vi "Build Win32 Wrappers.vi"(0 "only these wrappers":string[](array[string]), 11 "error in":errorcluster) -> (4 "wrappers":path[](array[path]), 15 "error out":errorcluster)   [LabVIEW 2020]
doc: "Creates or overwrites the Win32 wrapper VIs of the RemoteVI toolkit in source\\Win32 by VI scripting - one VI per DLL function, each listed in the wrapper specs constant on this diagram (wrapper name, template, DLL, function, parameter lines, link lines - see W32B Parse Spec.vi for the line format, and UI thread?). Each wrapper starts as a copy of its template in scripts\\Win32 Wrapper Templates (front panel, connector pane, icon, descriptions, helper nodes), then gets a Call Library Function Node placed, configured (stdcall, run in any thread - or in LabVIEW's UI thread when the spec's UI thread? is TRUE, typed parameters) and wired by VI Server - the one node AIXML cannot author. only these wrappers limits the run to the named wrapper VIs (empty = all); a wrapper that is loaded in LabVIEW (called by a running VI) cannot be overwritten. Run it from the IDE whenever a template or a spec changes. Paths are found relative to this VI, so the repository may live anywhere. The AIXML sources of the templates are in tools\\aixml\\Win32."
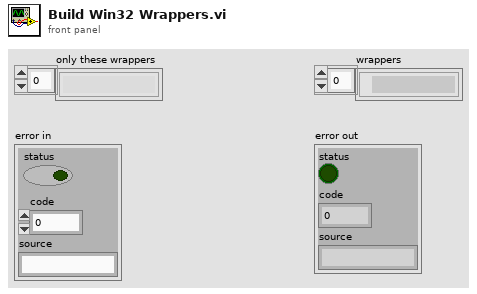
[diagram p1: front panel]
types:
  T1 = cluster{"wrapper name":string, "template":string, "library":path, "function":string, "parameters":string, "links":string, "UI thread?":bool}[]
  T2 = cluster{"function name":string, "library path":path, "parameter info":cluster{"Parameter Name":string, "Num Dimensions":i32, "Parameter Type":enum16{"Numeric", "Array", "String", "Waveform", "Digital Waveform", "Digital Table", "ActiveX", "Any", "Instance Data Pointer", "Void"}, "Numeric Type":enum16{"I8", "I16", "I32", "I64", "U8", "U16", "U32", "U64", "SGL", "DBL", "PTR INT", "PTR UINT"}, "Param Passing":enum16{"By Value", "Pointer To Value"}, "Array Passing":enum16{"Array Data Pointer", "Array Handle", "Array Handle Pointer"}, "String Passing":enum16{"C String Pointer", "Pascal String Pointer", "String Handle", "String Handle Pointer"}, "Adapt Format":enum16{"By Value", "Pointer To Value"}, "ActiveX Types":enum16{"ActiveX Variant Pointer", "IDispatch* Pointer", "IUnknown* Pointer"}, "Const (unused)":bool, "Minimum Size":string}[]}
  T3 = cluster{"CLFN terminal":i32, "control label":string, "node class":string, "node source?":bool}[]
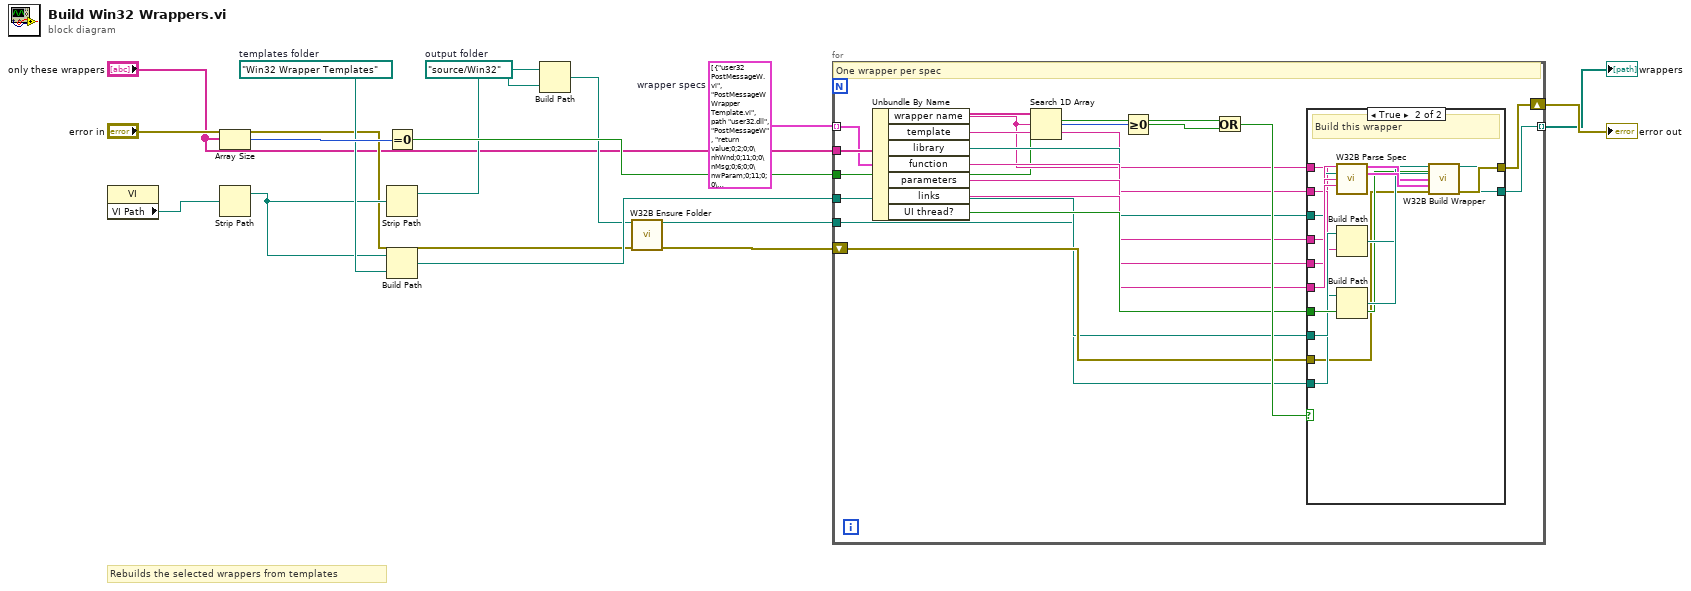
[diagram p0: block diagram]
diagram:
  w14 = T1 [{"wrapper name"="user32 PostMessageW.vi", "template"="PostMessageW Wrapper Template.vi", "library"=path "user32.dll", "function"="PostMessageW", "parameters"="return value;0;2;0;0\nhWnd;0;11;0;0\nMsg;0;6;0;0\nwParam;0;11;0;0\nlParam;0;10;0;0", "links"="2;error in (no error);;0\n3;error out;;0\n5;return value;;0\n6;hWnd;;0\n8;Msg;;0\n10;wParam;;0\n12;lParam;;0", "UI thread?"=FALSE}, {"wrapper name"="user32 ScreenToClient.vi", "template"="ScreenToClient Wrapper Template.vi", "library"=path "user32.dll", "function"="ScreenToClient", "parameters"="return value;0;2;0;0\nhWnd;0;11;0;0\nlpPoint;7;2;0;0", "links"="2;error in (no error);;0\n3;error out;;0\n5;return value;;0\n6;hWnd;;0\n8;;Bundler;1\n9;;Unbundler;0", "UI thread?"=FALSE}, {"wrapper name"="user32 FindWindowExW.vi", "template"="FindWindowExW Wrapper Template.vi", "library"=path "user32.dll", "function"="FindWindowExW", "parameters"="return value;0;11;0;0\nhWndParent;0;11;0;0\nhWndChildAfter;0;11;0;0\nlpszClass;1;5;0;0;1\nlpszWindow;1;5;0;0;1", "links"="2;error in;;0\n3;error out;;0\n5;hWnd;;0\n6;hWndParent;;0\n8;hWndChildAfter;;0\n10;lpszClass;;0\n12;lpszWindow;;0", "UI thread?"=FALSE}, {"wrapper name"="user32 GetWindowThreadProcessId.vi", "template"="GetWindowThreadProcessId Wrapper Template.vi", "library"=path "user32.dll", "function"="GetWindowThreadProcessId", "parameters"="return value;0;6;0;0\nhWnd;0;11;0;0\nlpdwProcessId;0;6;1;0", "links"="2;error in;;0\n3;error out;;0\n5;thread ID;;0\n6;hWnd;;0\n9;process ID;;0", "UI thread?"=FALSE}, {"wrapper name"="user32 IsWindowVisible.vi", "template"="IsWindowVisible Wrapper Template.vi", "library"=path "user32.dll", "function"="IsWindowVisible", "parameters"="return value;0;2;0;0\nhWnd;0;11;0;0", "links"="2;error in;;0\n3;error out;;0\n5;;Function;0\n6;hWnd;;0", "UI thread?"=FALSE}, {"wrapper name"="user32 IsIconic.vi", "template"="IsIconic Wrapper Template.vi", "library"=path "user32.dll", "function"="IsIconic", "parameters"="return value;0;2;0;0\nhWnd;0;11;0;0", "links"="2;error in;;0\n3;error out;;0\n5;;Function;0\n6;hWnd;;0", "UI thread?"=FALSE}, {"wrapper name"="user32 ShowWindow.vi", "template"="ShowWindow Wrapper Template.vi", "library"=path "user32.dll", "function"="ShowWindow", "parameters"="return value;0;2;0;0\nhWnd;0;11;0;0\nnCmdShow;0;2;0;0", "links"="2;error in;;0\n3;error out;;0\n5;return value;;0\n6;hWnd;;0\n8;nCmdShow;;0", "UI thread?"=FALSE}, {"wrapper name"="user32 GetWindowRect.vi", "template"="GetWindowRect Wrapper Template.vi", "library"=path "user32.dll", "function"="GetWindowRect", "parameters"="return value;0;2;0;0\nhWnd;0;11;0;0\nlpRect;7;2;0;0", "links"="2;error in;;0\n3;error out;;0\n5;return value;;0\n6;hWnd;;0\n8;;Bundler;1\n9;RECT;;0", "UI thread?"=FALSE}, {"wrapper name"="user32 GetClientRect.vi", "template"="GetClientRect Wrapper Template.vi", "library"=path "user32.dll", "function"="GetClientRect", "parameters"="return value;0;2;0;0\nhWnd;0;11;0;0\nlpRect;7;2;0;0", "links"="2;error in;;0\n3;error out;;0\n5;return value;;0\n6;hWnd;;0\n8;;Bundler;1\n9;RECT;;0", "UI thread?"=FALSE}, {"wrapper name"="user32 GetClassNameW.vi", "template"="GetClassNameW Wrapper Template.vi", "library"=path "user32.dll", "function"="GetClassNameW", "parameters"="return value;0;2;0;0\nhWnd;0;11;0;0\nlpClassName;1;5;0;0;1\nnMaxCount;0;2;0;0", "links"="2;error in;;0\n3;error out;;0\n5;return value;;0\n6;hWnd;;0\n8;;Unbundler;1\n9;;BuildArray;0\n10;nMaxCount;;0", "UI thread?"=FALSE}, {"wrapper name"="user32 GetWindowLongPtrW.vi", "template"="GetWindowLongPtrW Wrapper Template.vi", "library"=path "user32.dll", "function"="GetWindowLongPtrW", "parameters"="return value;0;10;0;0\nhWnd;0;11;0;0\nnIndex;0;2;0;0", "links"="2;error in;;0\n3;error out;;0\n5;return value;;0\n6;hWnd;;0\n8;nIndex;;0", "UI thread?"=FALSE}, {"wrapper name"="user32 SetWindowPos.vi", "template"="SetWindowPos Wrapper Template.vi", "library"=path "user32.dll", "function"="SetWindowPos", "parameters"="return value;0;2;0;0\nhWnd;0;11;0;0\nhWndInsertAfter;0;11;0;0\nX;0;2;0;0\nY;0;2;0;0\ncx;0;2;0;0\ncy;0;2;0;0\nuFlags;0;6;0;0", "links"="2;error in;;0\n3;error out;;0\n5;return value;;0\n6;hWnd;;0\n8;hWndInsertAfter;;0\n10;X;;0\n12;Y;;0\n14;cx;;0\n16;cy;;0\n18;uFlags;;0", "UI thread?"=FALSE}, {"wrapper name"="user32 SendMessageTimeoutW.vi", "template"="SendMessageTimeoutW Wrapper Template.vi", "library"=path "user32.dll", "function"="SendMessageTimeoutW", "parameters"="return value;0;10;0;0\nhWnd;0;11;0;0\nMsg;0;6;0;0\nwParam;0;11;0;0\nlParam;0;10;0;0\nfuFlags;0;6;0;0\nuTimeout;0;6;0;0\nlpdwResult;0;11;1;0", "links"="2;error in;;0\n3;error out;;0\n5;return value;;0\n6;hWnd;;0\n8;Msg;;0\n10;wParam;;0\n12;lParam;;0\n14;fuFlags;;0\n16;uTimeout;;0\n19;result;;0", "UI thread?"=FALSE}, {"wrapper name"="user32 GetDC.vi", "template"="GetDC Wrapper Template.vi", "library"=path "user32.dll", "function"="GetDC", "parameters"="return value;0;11;0;0\nhWnd;0;11;0;0", "links"="2;error in;;0\n3;error out;;0\n5;HDC;;0\n6;hWnd;;0", "UI thread?"=FALSE}, {"wrapper name"="user32 ReleaseDC.vi", "template"="ReleaseDC Wrapper Template.vi", "library"=path "user32.dll", "function"="ReleaseDC", "parameters"="return value;0;2;0;0\nhWnd;0;11;0;0\nhDC;0;11;0;0", "links"="2;error in;;0\n3;error out;;0\n5;return value;;0\n6;hWnd;;0\n8;hDC;;0", "UI thread?"=FALSE}, {"wrapper name"="kernel32 GetCurrentProcessId.vi", "template"="GetCurrentProcessId Wrapper Template.vi", "library"=path "kernel32.dll", "function"="GetCurrentProcessId", "parameters"="return value;0;6;0;0", "links"="2;error in;;0\n3;error out;;0\n5;process ID;;0", "UI thread?"=FALSE}, {"wrapper name"="gdi32 CreateCompatibleDC.vi", "template"="CreateCompatibleDC Wrapper Template.vi", "library"=path "gdi32.dll", "function"="CreateCompatibleDC", "parameters"="return value;0;11;0;0\nhdc;0;11;0;0", "links"="2;error in;;0\n3;error out;;0\n5;HDC;;0\n6;hdc;;0", "UI thread?"=FALSE}, {"wrapper name"="gdi32 CreateCompatibleBitmap.vi", "template"="CreateCompatibleBitmap Wrapper Template.vi", "library"=path "gdi32.dll", "function"="CreateCompatibleBitmap", "parameters"="return value;0;11;0;0\nhdc;0;11;0;0\ncx;0;2;0;0\ncy;0;2;0;0", "links"="2;error in;;0\n3;error out;;0\n5;HBITMAP;;0\n6;hdc;;0\n8;cx;;0\n10;cy;;0", "UI thread?"=FALSE}, {"wrapper name"="gdi32 SelectObject.vi", "template"="SelectObject Wrapper Template.vi", "library"=path "gdi32.dll", "function"="SelectObject", "parameters"="return value;0;11;0;0\nhdc;0;11;0;0\nh;0;11;0;0", "links"="2;error in;;0\n3;error out;;0\n5;previous object;;0\n6;hdc;;0\n8;h;;0", "UI thread?"=FALSE}, {"wrapper name"="gdi32 GetDIBits.vi", "template"="GetDIBits Wrapper Template.vi", "library"=path "gdi32.dll", "function"="GetDIBits", "parameters"="return value;0;2;0;0\nhdc;0;11;0;0\nhbm;0;11;0;0\nstart;0;6;0;0\ncLines;0;6;0;0\nlpvBits;1;6;0;0;1\nlpbmi;7;2;0;0\nusage;0;6;0;0", "links"="2;error in;;0\n3;error out;;0\n5;return value;;0\n6;hdc;;0\n8;hbm;;0\n10;start;;0\n12;cLines;;0\n14;lpvBits;;0\n15;lpvBits out;;0\n16;lpbmi;;0\n18;usage;;0", "UI thread?"=FALSE}, {"wrapper name"="gdi32 DeleteObject.vi", "template"="DeleteObject Wrapper Template.vi", "library"=path "gdi32.dll", "function"="DeleteObject", "parameters"="return value;0;2;0;0\nho;0;11;0;0", "links"="2;error in;;0\n3;error out;;0\n5;return value;;0\n6;ho;;0", "UI thread?"=FALSE}, {"wrapper name"="gdi32 DeleteDC.vi", "template"="DeleteDC Wrapper Template.vi", "library"=path "gdi32.dll", "function"="DeleteDC", "parameters"="return value;0;2;0;0\nhdc;0;11;0;0", "links"="2;error in;;0\n3;error out;;0\n5;return value;;0\n6;hdc;;0", "UI thread?"=FALSE}, {"wrapper name"="user32 PrintWindow.vi", "template"="PrintWindow Wrapper Template.vi", "library"=path "user32.dll", "function"="PrintWindow", "parameters"="return value;0;2;0;0\nhwnd;0;11;0;0\nhdcBlt;0;11;0;0\nnFlags;0;6;0;0", "links"="2;error in;;0\n3;error out;;0\n5;return value;;0\n6;hwnd;;0\n8;hdcBlt;;0\n10;nFlags;;0", "UI thread?"=FALSE}, {"wrapper name"="user32 SetWindowLongPtrW.vi", "template"="SetWindowLongPtrW Wrapper Template.vi", "library"=path "user32.dll", "function"="SetWindowLongPtrW", "parameters"="return value;0;10;0;0\nhWnd;0;11;0;0\nnIndex;0;2;0;0\ndwNewLong;0;10;0;0", "links"="2;error in;;0\n3;error out;;0\n5;return value;;0\n6;hWnd;;0\n8;nIndex;;0\n10;dwNewLong;;0", "UI thread?"=FALSE}, {"wrapper name"="user32 SetLayeredWindowAttributes.vi", "template"="SetLayeredWindowAttributes Wrapper Template.vi", "library"=path "user32.dll", "function"="SetLayeredWindowAttributes", "parameters"="return value;0;2;0;0\nhwnd;0;11;0;0\ncrKey;0;6;0;0\nbAlpha;0;4;0;0\ndwFlags;0;6;0;0", "links"="2;error in;;0\n3;error out;;0\n5;return value;;0\n6;hwnd;;0\n8;crKey;;0\n10;bAlpha;;0\n12;dwFlags;;0", "UI thread?"=FALSE}, {"wrapper name"="user32 GetCursorPos.vi", "template"="GetCursorPos Wrapper Template.vi", "library"=path "user32.dll", "function"="GetCursorPos", "parameters"="return value;0;2;0;0\nlpPoint;7;2;0;0", "links"="2;error in;;0\n3;error out;;0\n5;return value;;0\n6;;Bundler;1\n7;;Unbundler;0", "UI thread?"=FALSE}, {"wrapper name"="user32 GetKeyboardState.vi", "template"="GetKeyboardState Wrapper Template.vi", "library"=path "user32.dll", "function"="GetKeyboardState", "parameters"="return value;0;2;0;0\nlpKeyState;1;4;0;0;1", "links"="2;error in;;0\n3;error out;;0\n5;return value;;0\n6;;Unbundler;1\n7;;BuildArray;0", "UI thread?"=TRUE}, {"wrapper name"="user32 SetKeyboardState.vi", "template"="SetKeyboardState Wrapper Template.vi", "library"=path "user32.dll", "function"="SetKeyboardState", "parameters"="return value;0;2;0;0\nlpKeyState;1;4;0;0;1", "links"="2;error in;;0\n3;error out;;0\n5;return value;;0\n6;;Unbundler;1\n7;;BuildArray;0", "UI thread?"=TRUE}, {"wrapper name"="user32 GetGUIThreadInfo.vi", "template"="GetGUIThreadInfo Wrapper Template.vi", "library"=path "user32.dll", "function"="GetGUIThreadInfo", "parameters"="return value;0;2;0;0\nidThread;0;6;0;0\npgui;1;6;0;0;1", "links"="2;error in;;0\n3;error out;;0\n5;return value;;0\n6;thread ID;;0\n8;;Unbundler;1\n9;;BuildArray;0", "UI thread?"=FALSE}, {"wrapper name"="user32 GetSysColor.vi", "template"="GetSysColor Wrapper Template.vi", "library"=path "user32.dll", "function"="GetSysColor", "parameters"="return value;0;6;0;0\nnIndex;0;2;0;0", "links"="2;error in;;0\n3;error out;;0\n5;color;;0\n6;nIndex;;0", "UI thread?"=FALSE}, {"wrapper name"="user32 GetWindow.vi", "template"="GetWindow Wrapper Template.vi", "library"=path "user32.dll", "function"="GetWindow", "parameters"="return value;0;11;0;0\nhWnd;0;11;0;0\nuCmd;0;6;0;0", "links"="2;error in;;0\n3;error out;;0\n5;window;;0\n6;hWnd;;0\n8;uCmd;;0", "UI thread?"=FALSE}, {"wrapper name"="user32 GetAncestor.vi", "template"="GetAncestor Wrapper Template.vi", "library"=path "user32.dll", "function"="GetAncestor", "parameters"="return value;0;11;0;0\nhwnd;0;11;0;0\ngaFlags;0;6;0;0", "links"="2;error in;;0\n3;error out;;0\n5;ancestor;;0\n6;hwnd;;0\n8;gaFlags;;0", "UI thread?"=FALSE}, {"wrapper name"="user32 IsWindowEnabled.vi", "template"="IsWindowEnabled Wrapper Template.vi", "library"=path "user32.dll", "function"="IsWindowEnabled", "parameters"="return value;0;2;0;0\nhWnd;0;11;0;0", "links"="2;error in;;0\n3;error out;;0\n5;;Function;0\n6;hWnd;;0", "UI thread?"=FALSE}, {"wrapper name"="user32 GetWindowTextW.vi", "template"="GetWindowTextW Wrapper Template.vi", "library"=path "user32.dll", "function"="GetWindowTextW", "parameters"="return value;0;2;0;0\nhWnd;0;11;0;0\nlpString;1;5;0;0;1\nnMaxCount;0;2;0;0", "links"="2;error in;;0\n3;error out;;0\n5;return value;;0\n6;hWnd;;0\n8;;Unbundler;1\n9;;BuildArray;0\n10;nMaxCount;;0", "UI thread?"=FALSE}, {"wrapper name"="user32 ChildWindowFromPointEx.vi", "template"="ChildWindowFromPointEx Wrapper Template.vi", "library"=path "user32.dll", "function"="ChildWindowFromPointEx", "parameters"="return value;0;11;0;0\nhwnd;0;11;0;0\npt;0;7;0;0\nflags;0;6;0;0", "links"="2;error in;;0\n3;error out;;0\n5;child;;0\n6;hwnd;;0\n8;pt;;0\n10;flags;;0", "UI thread?"=FALSE}, {"wrapper name"="gdi32 CreateRectRgn.vi", "template"="CreateRectRgn Wrapper Template.vi", "library"=path "gdi32.dll", "function"="CreateRectRgn", "parameters"="return value;0;11;0;0\nx1;0;2;0;0\ny1;0;2;0;0\nx2;0;2;0;0\ny2;0;2;0;0", "links"="2;error in;;0\n3;error out;;0\n5;HRGN;;0\n6;x1;;0\n8;y1;;0\n10;x2;;0\n12;y2;;0", "UI thread?"=FALSE}, {"wrapper name"="user32 SetWindowRgn.vi", "template"="SetWindowRgn Wrapper Template.vi", "library"=path "user32.dll", "function"="SetWindowRgn", "parameters"="return value;0;2;0;0\nhWnd;0;11;0;0\nhRgn;0;11;0;0\nbRedraw;0;2;0;0", "links"="2;error in;;0\n3;error out;;0\n5;return value;;0\n6;hWnd;;0\n8;hRgn;;0\n10;bRedraw;;0", "UI thread?"=FALSE}, {"wrapper name"="gdi32 BitBlt.vi", "template"="BitBlt Wrapper Template.vi", "library"=path "gdi32.dll", "function"="BitBlt", "parameters"="return value;0;2;0;0\nhdc;0;11;0;0\nx;0;2;0;0\ny;0;2;0;0\ncx;0;2;0;0\ncy;0;2;0;0\nhdcSrc;0;11;0;0\nx1;0;2;0;0\ny1;0;2;0;0\nrop;0;6;0;0", "links"="2;error in;;0\n3;error out;;0\n5;return value;;0\n6;hdc;;0\n8;x;;0\n10;y;;0\n12;cx;;0\n14;cy;;0\n16;hdcSrc;;0\n18;x1;;0\n20;y1;;0\n22;rop;;0", "UI thread?"=FALSE}, {"wrapper name"="bcrypt BCryptGenRandom.vi", "template"="BCryptGenRandom Wrapper Template.vi", "library"=path "bcrypt.dll", "function"="BCryptGenRandom", "parameters"="return value;0;2;0;0\nhAlgorithm;0;11;0;0\npbBuffer;1;4;0;0;1\ncbBuffer;0;6;0;0\ndwFlags;0;6;0;0", "links"="2;error in;;0\n3;error out;;0\n5;return value;;0\n6;hAlgorithm;;0\n8;;Unbundler;1\n9;;BuildArray;0\n10;byte count;;0\n12;dwFlags;;0", "UI thread?"=FALSE}, {"wrapper name"="kernel32 OpenProcess.vi", "template"="OpenProcess Wrapper Template.vi", "library"=path "kernel32.dll", "function"="OpenProcess", "parameters"="return value;0;11;0;0\ndwDesiredAccess;0;6;0;0\nbInheritHandle;0;2;0;0\ndwProcessId;0;6;0;0", "links"="2;error in;;0\n3;error out;;0\n5;HANDLE;;0\n6;dwDesiredAccess;;0\n8;bInheritHandle;;0\n10;process ID;;0", "UI thread?"=FALSE}, {"wrapper name"="kernel32 QueryFullProcessImageNameW.vi", "template"="QueryFullProcessImageNameW Wrapper Template.vi", "library"=path "kernel32.dll", "function"="QueryFullProcessImageNameW", "parameters"="return value;0;2;0;0\nhProcess;0;11;0;0\ndwFlags;0;6;0;0\nlpExeName;1;5;0;0;1\nlpdwSize;0;6;1;0", "links"="2;error in;;0\n3;error out;;0\n5;return value;;0\n6;hProcess;;0\n8;dwFlags;;0\n10;;Unbundler;1\n11;;BuildArray;0\n12;size;;0", "UI thread?"=FALSE}, {"wrapper name"="kernel32 CloseHandle.vi", "template"="CloseHandle Wrapper Template.vi", "library"=path "kernel32.dll", "function"="CloseHandle", "parameters"="return value;0;2;0;0\nhObject;0;11;0;0", "links"="2;error in;;0\n3;error out;;0\n5;return value;;0\n6;hObject;;0", "UI thread?"=FALSE}, {"wrapper name"="user32 IsWindow.vi", "template"="IsWindow Wrapper Template.vi", "library"=path "user32.dll", "function"="IsWindow", "parameters"="return value;0;2;0;0\nhWnd;0;11;0;0", "links"="2;error in;;0\n3;error out;;0\n5;;Function;0\n6;hWnd;;0", "UI thread?"=FALSE}, {"wrapper name"="kernel32 GetCurrentThreadId.vi", "template"="GetCurrentThreadId Wrapper Template.vi", "library"=path "kernel32.dll", "function"="GetCurrentThreadId", "parameters"="return value;0;6;0;0", "links"="2;error in;;0\n3;error out;;0\n5;thread ID;;0", "UI thread?"=TRUE}, {"wrapper name"="user32 AttachThreadInput.vi", "template"="AttachThreadInput Wrapper Template.vi", "library"=path "user32.dll", "function"="AttachThreadInput", "parameters"="return value;0;2;0;0\nidAttach;0;6;0;0\nidAttachTo;0;6;0;0\nfAttach;0;2;0;0", "links"="2;error in;;0\n3;error out;;0\n5;return value;;0\n6;idAttach;;0\n8;idAttachTo;;0\n10;fAttach;;0", "UI thread?"=TRUE}, {"wrapper name"="LabVIEW LVImageDataToPNGByteArray.vi", "template"="LVImageDataToPNGByteArray Wrapper Template.vi", "library"=path "LabVIEW", "function"="LVImageDataToPNGByteArray", "parameters"="return value;9;0;0;0\npngOutput;1;4;0;0;1;2\ncompression;0;2;0;0\nimageWidth;0;6;0;0\nimageHeight;0;6;0;0\ndepth;0;1;0;0\nimageBuf;1;4;0;0;1;0\ncolorTable;1;2;0;0;1;0\ncolorTableSize;0;2;0;0", "links"="2;error in;;0\n3;error out;;0\n7;png data;;0\n8;compression;;0\n10;width;;0\n12;height;;0\n14;depth;;0\n16;imageBuf;;0\n18;colorTable;;0\n20;colorTableSize;;0", "UI thread?"=FALSE}]  # wrapper specs
  w12 = path "Win32 Wrapper Templates"  # templates folder
  w8 = path "source/Win32"  # output folder
  # "Rebuilds the selected wrappers from templates"
  n1 = property class="VI"() -> ("VI Path"=w5:path)  [unwired: 2 in, 2 out]
  n2 = Array Size(array="only these wrappers") -> (size(s)=w15:i32)
  n3 = Strip Path(path=w5) -> (stripped path=w6:path)  [unwired: 1 out]
  n4 = Equal To 0?(x=w15) -> (x = 0?=w16:bool)
  n5 = Strip Path(path=w6) -> (stripped path=w7:path)  [unwired: 1 out]
  n6 = Build Path(base path=w6, name or relative path=w12) -> (appended path=w13:path)
  n7 = Build Path(base path=w7, name or relative path=w8) -> (appended path=w9:path)
  n8 = call "W32B Ensure Folder.vi"("folder"=w9, "error in"="error in") -> ("folder out"=w10:path, "error out"=w11:errorcluster)  [unwired: 12 in]
  n9 = for {
    tunnel: w14 -> [w17] mode=indexing
    tunnel: "only these wrappers" -> [w20]
    tunnel: w16 -> [w21]
    tunnel: w13 -> [w19]
    tunnel: w10 -> [w18]
    shift-right: [w23] -> w4
    shift-left: w11 -> [w22]
    tunnel: [w34] -> w3 mode=indexing
    # "One wrapper per spec"
    n10 = Unbundle By Name(w17) -> ("wrapper name"=w24:string, "template"=w25:string, "library"=w26:path, "function"=w27:string, "parameters"=w28:string, "links"=w29:string, "UI thread?"=w30:bool)
    n11 = Search 1D Array(1D array=w20, element=w24) -> (index of element=w31:i32)  [unwired: 1 in]
    n12 = Greater Or Equal To 0?(x=w31) -> (x >= 0?=w32:bool)
    n13 = Or(x=w21, y=w32) -> (x .or. y?=w33:bool)
    n14 = case shown="True" w33 {
      tunnel: w24 -> [_ w37]
      tunnel: w25 -> [_ w38]
      tunnel: w26 -> [_ w39]
      tunnel: w27 -> [_ w40]
      tunnel: w28 -> [_ w41]
      tunnel: w29 -> [_ w42]
      tunnel: w30 -> [_ w45]
      tunnel: w19 -> [_ w44]
      tunnel: w22 -> [w35 w36]
      tunnel: w18 -> [_ w43]
      tunnel: [w35 w51] -> w23
      tunnel: [_ w50] -> w34
      frame False {
        # "Not selected - skip"
      }
      frame True {
        # "Build this wrapper"
        n15 = call "W32B Parse Spec.vi"("function name"=w40, "library path"=w39, "parameters"=w41, "links"=w42) -> ("CLFN"=w48:T2, "links out"=w49:T3)  [unwired: 9 in, 1 out]
        n16 = Build Path(base path=w44, name or relative path=w38) -> (appended path=w46:path)
        n17 = Build Path(base path=w43, name or relative path=w37) -> (appended path=w47:path)
        n18 = call "W32B Build Wrapper.vi"("template path"=w46, "run in UI thread?"=w45, "target path"=w47, "CLFN"=w48, "links"=w49, "error in"=w36) -> ("wrapper path"=w50:path, "error out"=w51:errorcluster)  [unwired: 8 in]
      }
    }
  }
  "wrappers" <- w3
  "error out" <- w4
